vi "FX_WriteWord.vi"(8 "error in (no error)":errorcluster, 9 "Value":u16, 10 "Device":string, 11 "PLC Conn":refnum<visa-resource-name>) -> (2 "error out":errorcluster, 3 "PLC Conn out":refnum<visa-resource-name>)   [LabVIEW 2018]
doc: "Use this template to build a VI to use as a subVI."
panel:
  # "說明：寫一個 D，低位元組在前。"
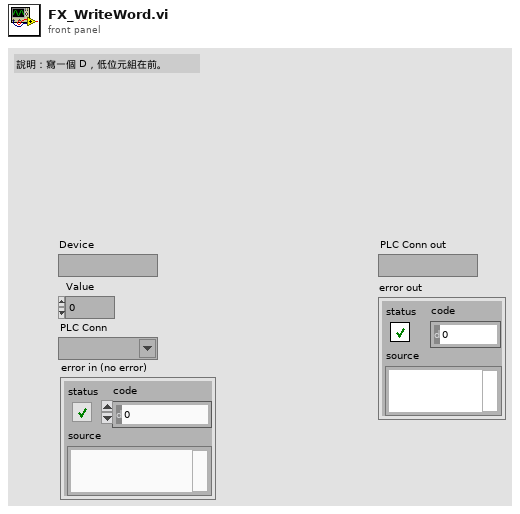
[diagram p1: front panel]
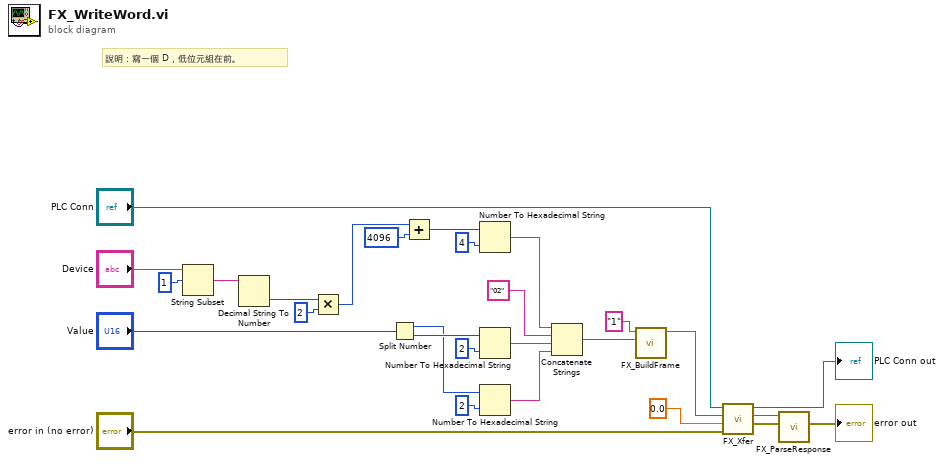
[diagram p0: block diagram]
diagram:
  # "說明：寫一個 D，低位元組在前。"
  n1 = String Subset(string="Device", offset (0)=1) -> (substring=w24:string)  [unwired: 1 in]
  n2 = Decimal String To Number(string=w24) -> (number=w23:i32)  [unwired: 2 in, 1 out]
  n3 = Multiply(x=w23, y=2) -> (x*y=w21:i32)
  n4 = Split Number(x="Value") -> (hi(x)=w15:u8, lo(x)=w17:u8)
  n5 = Add(x=w21, y=4096) -> (x+y=w19:i32)
  n6 = Number To Hexadecimal String(1:i16 4 ("width (-)"), 2:w19) -> (0:w13:string)
  n7 = Number To Hexadecimal String(1:i16 2 ("width (-)"), 2:w17) -> (0:w11:string)
  n8 = Number To Hexadecimal String(1:i16 2 ("width (-)"), 2:w15) -> (0:w10:string)
  n9 = Concatenate Strings(w13, "02", w11, w10) -> (w9:string)
  n10 = call "FX_BuildFrame.vi"("Content"=w9, "Command"="1") -> ("Frame"=w8:string)  [unwired: 9 in]
  n11 = call "FX_Xfer.vi"("error in (no error)"="error in (no error)", "Data Chars"=0.0, "TX"=w8, "PLC Conn"="PLC Conn") -> ("error out"=w3:errorcluster, "RX"=w4:string, "PLC Conn out"=→"PLC Conn out":refnum<visa-resource-name>)  [unwired: 5 in]
  n12 = call "FX_ParseResponse.vi"("error in (no error)"=w3, "RX"=w4) -> ("error out"=→"error out":errorcluster)  [unwired: 8 in, 1 out]
